vi "ACW Limiter.vi"(0 "ACW Test Frequency(Hz)":u8(ring)=1 items=["50", "60"], 1 "ACW Test Time(S)":sgl=0.5 min=0.5 max=999.9 format="%.1f", 2 "ACW HI SET current value(mA)":sgl=42.0 min=0.001 max=42 format="%.3f", 3 "ACW LO SET current value(mA)":sgl min=0 max=41.9 format="%.3f", 4 "Ramp Time":sgl=0.1 min=0.1 max=999.9 format="%.1f", 5 "ACW voltage(kV)":sgl=0.1 min=0.1 max=5 format="%.3f") -> (14 "ACW voltage(kV)":string, 15 "Ramp Time":string, 16 "ACW LO SET current value(mA)":string, 17 "ACW HI SET current value(mA)":string, 18 "ACW Test Time(S)":string, 19 "ACW Test Frequency(Hz)":string)   [LabVIEW 2021]
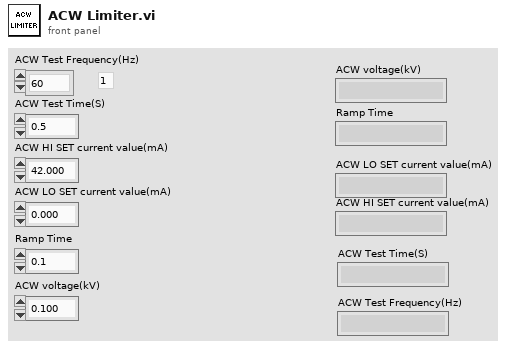
[diagram p1: front panel]
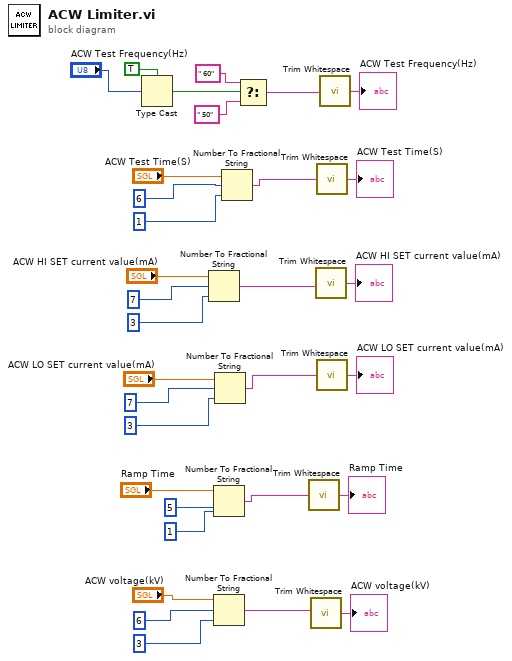
[diagram p0: block diagram]
diagram:
  n1 = Type Cast(type=TRUE, x="ACW Test Frequency(Hz)") -> (*(type *) &x=w28:bool)
  n2 = Number To Fractional String(number="ACW HI SET current value(mA)", width (-)=i16 7, precision (6)=i16 3) -> (F-format string=w10:string)  [unwired: 1 in]
  n3 = Number To Fractional String(number="Ramp Time", width (-)=i16 5, precision (6)=i16 1) -> (F-format string=w8:string)  [unwired: 1 in]
  n4 = Number To Fractional String(number="ACW voltage(kV)", width (-)=i16 6, precision (6)=i16 3) -> (F-format string=w7:string)  [unwired: 1 in]
  n5 = Number To Fractional String(number="ACW LO SET current value(mA)", width (-)=i16 7, precision (6)=i16 3) -> (F-format string=w9:string)  [unwired: 1 in]
  n6 = Number To Fractional String(number="ACW Test Time(S)", width (-)=i16 6, precision (6)=i16 1 ("width (-)")) -> (F-format string=w11:string)  [unwired: 1 in]
  n7 = Select(t=" 60", s=w28, f=" 50") -> (s? t:f=w12:string)
  n8 = call <vilib>:"Trim Whitespace.vi"("string"=w8) -> ("trimmed string"=→"Ramp Time":string)  [unwired: 1 in]
  n9 = call <vilib>:"Trim Whitespace.vi"("string"=w7) -> ("trimmed string"=→"ACW voltage(kV)":string)  [unwired: 1 in]
  n10 = call <vilib>:"Trim Whitespace.vi"("string"=w10) -> ("trimmed string"=→"ACW HI SET current value(mA)":string)  [unwired: 1 in]
  n11 = call <vilib>:"Trim Whitespace.vi"("string"=w11) -> ("trimmed string"=→"ACW Test Time(S)":string)  [unwired: 1 in]
  n12 = call <vilib>:"Trim Whitespace.vi"("string"=w9) -> ("trimmed string"=→"ACW LO SET current value(mA)":string)  [unwired: 1 in]
  n13 = call <vilib>:"Trim Whitespace.vi"("string"=w12) -> ("trimmed string"=→"ACW Test Frequency(Hz)":string)  [unwired: 1 in]
